vi "Read Return Header.vi"(8 "error in (no error)":errorcluster, 10 "Name":string, 11 "WebSocket in":refnum<class "WebSocket.lvclass">) -> (0 "error out":errorcluster, 1 "Found?":bool, 2 "Value":string, 3 "WebSocket out":refnum<class "WebSocket.lvclass">)   [LabVIEW 2013, in "WebSockets.lvlib" / "WebSocket.lvclass"]
doc: "Retrieves a named header from the received HTTP handshaking data."
uses:
  WebSocket.lvclass
  WebSocket.lvclass/WebSocket.ctl
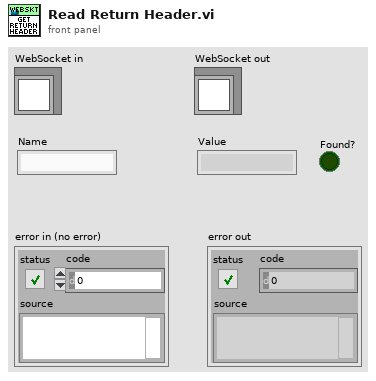
[diagram p1: front panel]
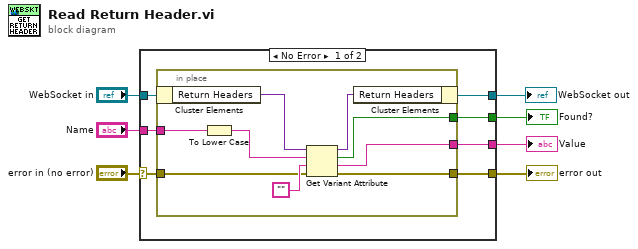
[diagram p0: block diagram]
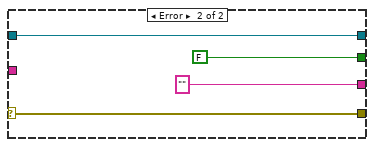
[diagram p2: hidden frame]
diagram:
  n1 = case shown="No Error" "error in (no error)" {
    selector: "error in (no error)" -> [w12 w27]
    tunnel: [w14 ""] -> w7
    tunnel: "Name" -> [w13 _]
    tunnel: "WebSocket in" -> [w9 w26]
    tunnel: [w8 w26] -> w2
    tunnel: [w11 w27] -> w4
    tunnel: [w10 FALSE] -> w3
    frame No Error {
      n2 = in-place {
        in-place-border: [w23] -> w14
        in-place-border: w13 -> [w21]
        in-place-border: w12 -> [w20]
        in-place-border: [w19] -> w11
        in-place-border: [w18] -> w10
        n3 = in-place-cluster #1(w9) -> ("Return Headers"=w17:variant)
        n4 = To Lower Case(string=w21) -> (all lower case string=w15:string)
        n5 = Get Variant Attribute(Variant=w17, name=w15, default value (empty Variant)="", error in=w20) -> (duplicate Variant=w16:variant, found=w18:bool, value=w23:string, error out=w19:errorcluster)
        n6 = in-place-cluster #1("Return Headers"=w16) -> (w8:refnum<class "WebSocket.lvclass">)
      }
    }
    frame Error {
    }
  }
  "Value" <- w7
  "error out" <- w4
  "Found?" <- w3
  "WebSocket out" <- w2
